vi "FuncVI-QueuePut.vi"(5 "InstanceRef":T2, 9 "arg list":T1[](array[typedef]) {"num" format="%.2f"}) -> (0 "error out":bool, 3 "result":T1 {"num" format="%.2f"})   [LabVIEW 2021]
doc: "::: CalcExpress Toolkit :::\nCopyright (c) 2000-2026 Konstantin Shifershteyn. All rights reserved."
uses:
  cetypes.llb/CalcExpress Function Argument Info.ctl
  cetypes.llb/CalcExpress Instance RefNum.ctl
panel:
  in  "max arg num":i32=4
  in  "min arg num":i32=2
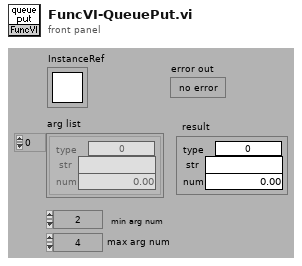
[diagram p1: front panel]
types:
  T1 = typedef "CalcExpress Function Argument Info.ctl" = cluster{"type":u32, "str":string, "num":dbl}
  T2 = typedef "CalcExpress Instance RefNum.ctl" = refnum<k1>
  T3 = cluster{"index":i32, "data type":enum32{"String", "DBL Number", "identifier", "1D Array of DBL", "2D Array of DBL", "CDB Number", "1D Array of CDB", "2D Array of CDB", "1D Array of String", "2D Array of String", "Unknown data type"}, "default num":dbl, "default str":string}[]
  T4 = enum32{"String", "DBL Number", "identifier", "1D Array of DBL", "2D Array of DBL", "CDB Number", "1D Array of CDB", "2D Array of CDB", "1D Array of String", "2D Array of String", "Unknown data type"}
  T5 = cluster{"data type":enum32{"String", "DBL Number", "identifier", "1D Array of DBL", "2D Array of DBL", "CDB Number", "1D Array of CDB", "2D Array of CDB", "1D Array of String", "2D Array of String", "Unknown data type"}, string, dbl}
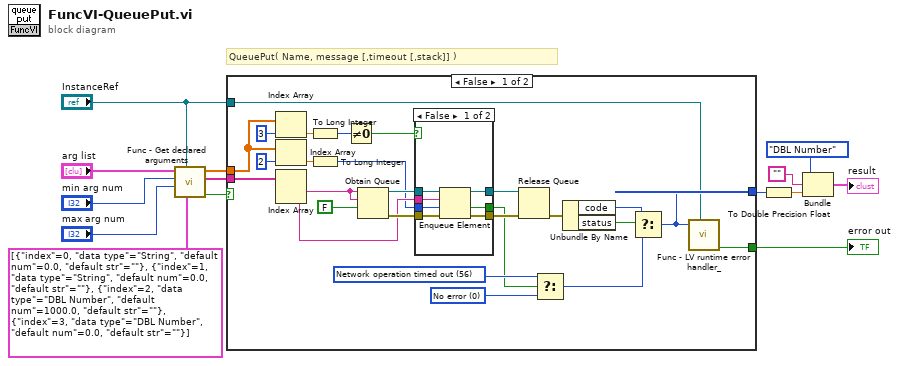
[diagram p0: block diagram]
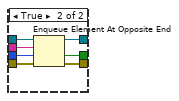
[diagram p2: hidden frame]
diagram:
  # "QueuePut( Name, message [,timeout [,stack]] )"
  n1 = call "Func - Get declared arguments.vi"("arg descriptors"=T3 [{"index"=0, "data type"=enum."String", "default num"=0.0, "default str"=""}, {"index"=1, "data type"=enum."String", "default num"=0.0, "default str"=""}, {"index"=2, "data type"=enum."DBL Number", "default num"=1000.0, "default str"=""}, {"index"=3, "data type"=enum."DBL Number", "default num"=0.0, "default str"=""}], "InstanceRef"="InstanceRef", "max arg num"="max arg num", "min arg num"="min arg num", "arg list"="arg list") -> ("error out"=w4:bool, "str list"=w13:string[], "num list"=w5:dbl[])  [unwired: 3 in, 1 out]
  n2 = case shown="False" w4 {
    selector: w4 -> [_ w55]
    tunnel: w13 -> [w40 _]
    tunnel: "InstanceRef" -> [w39 _]
    tunnel: [w27 _] -> w7
    tunnel: w5 -> [w36 _]
    tunnel: [w26 w55] -> w3
    frame False {
      w28 = 0 items=["No error", "Argument error", "Memory is full", "Out of zone", "End of file", "File already open", "Generic file I/O error", "File not found", "File permission error", "Disk is full", "Duplicate path", "Too many files open", "System feature not enabled", "Resource file not found", "Cannot add resource", "Resource not found", "Image not found", "Image memory error", "Pen does not exist", "Config type invalid", "Config token not found", "Config parse error", "Config memory error", "Bad external code format", "Bad external code offset", "External code not present", "Null window", "Destroy window error", "Null menu", "Print aborted", "Bad print record", "Print driver error", "Windows error during printing", "Memory error during printing", "Print dialog error", "Generic print error", "Invalid device refnum", "Device not found", "Device parameter error", "Device unit error", "Cannot open device", "Device call aborted", "Generic error", "Cancelled by user", "Object ID too low", "Object ID too high", "Object not in heap", "Unknown heap", "Unknown object (invalid DefProc)", "Unknown object (DefProc not in table)", "Message out of range", "Invalid (null) method", "Unknown message", "Manager call not supported", "Bad address", "Network operation in progress", "Network operation timed out", "Connection is busy", "Network attribute not supported", "Network error", "Address in use", "System out of memory", "Connection aborted", "Connection refused", "Not connected", "Already connected", "Connection closed", "Initialization error (interapplication manager)", "Bad occurrence", "Wait on unbound occurrence handler", "Occurrence queue overflow", "Datalog type conflict", "Unused", "Unrecognized type (interapplication manager)", "Memory corrupt", "Failed to make temporary DLL", "Old CIN version", "Drag socket not found", "Failed to load drop-object", "Failed to register OLE object", "Failed to release OLE object", "Format specifier type mismatch", "Unknown format specifier", "Too few format specifiers", "Too many format specifiers", "Scan failed", "Newer CIN version", "OLE Convert", "Runtime menu error", "Password tampered", "Unknown error code"]
      w31 = 56 items=["No error", "Argument error", "Memory is full", "Out of zone", "End of file", "File already open", "Generic file I/O error", "File not found", "File permission error", "Disk is full", "Duplicate path", "Too many files open", "System feature not enabled", "Resource file not found", "Cannot add resource", "Resource not found", "Image not found", "Image memory error", "Pen does not exist", "Config type invalid", "Config token not found", "Config parse error", "Config memory error", "Bad external code format", "Bad external code offset", "External code not present", "Null window", "Destroy window error", "Null menu", "Print aborted", "Bad print record", "Print driver error", "Windows error during printing", "Memory error during printing", "Print dialog error", "Generic print error", "Invalid device refnum", "Device not found", "Device parameter error", "Device unit error", "Cannot open device", "Device call aborted", "Generic error", "Cancelled by user", "Object ID too low", "Object ID too high", "Object not in heap", "Unknown heap", "Unknown object (invalid DefProc)", "Unknown object (DefProc not in table)", "Message out of range", "Invalid (null) method", "Unknown message", "Manager call not supported", "Bad address", "Network operation in progress", "Network operation timed out", "Connection is busy", "Network attribute not supported", "Network error", "Address in use", "System out of memory", "Connection aborted", "Connection refused", "Not connected", "Already connected", "Connection closed", "Initialization error (interapplication manager)", "Bad occurrence", "Wait on unbound occurrence handler", "Occurrence queue overflow", "Datalog type conflict", "Unused", "Unrecognized type (interapplication manager)", "Memory corrupt", "Failed to make temporary DLL", "Old CIN version", "Drag socket not found", "Failed to load drop-object", "Failed to register OLE object", "Failed to release OLE object", "Format specifier type mismatch", "Unknown format specifier", "Too few format specifiers", "Too many format specifiers", "Scan failed", "Newer CIN version", "OLE Convert", "Runtime menu error", "Password tampered", "Unknown error code"]
      n3 = Index Array(array=w36, index=3) -> (element=w35:dbl)
      n4 = Index Array(array=w36, index=2) -> (element=w34:dbl)
      n5 = Index Array(array=w40) -> (element #1=w18:string, element #2=w17:string)  [unwired: 2 in]
      n6 = To Long Integer(number=w35) -> (32bit integer=w33:i32)
      n7 = To Long Integer(number=w34) -> (32bit integer=w16:i32)
      n8 = Not Equal To 0?(x=w33) -> (x != 0?=w20:bool)
      n9 = Obtain Queue(name (unnamed)=w18, element data type=w18, create if not found? (T)=FALSE) -> (queue out=w25:refnum<queue>, error out=w23:errorcluster)  [unwired: 2 in, 1 out]
      n10 = case shown="False" w20 {
        tunnel: w25 -> [w47 w54]
        tunnel: [w46 w51] -> w24
        tunnel: w23 -> [w45 w53]
        tunnel: [w44 w52] -> w22
        tunnel: [w43 w50] -> w19
        tunnel: w17 -> [w42 w49]
        tunnel: w16 -> [w41 w48]
        frame False {
          n11 = Enqueue Element(queue=w47, element=w42, timeout in ms (-1)=w41, error in (no error)=w45) -> (queue out=w46:refnum<queue>, timed out?=w43:bool, error out=w44:errorcluster)
        }
        frame True {
          n12 = Enqueue Element At Opposite End(queue=w54, element=w49, timeout in ms (-1)=w48, error in (no error)=w53) -> (queue out=w51:refnum<queue>, timed out?=w50:bool, error out=w52:errorcluster)
        }
      }
      n13 = Release Queue(queue=w24, error in (no error)=w22) -> (error out=w15:errorcluster)  [unwired: 1 in, 2 out]
      n14 = Select(t=w31, s=w19, f=w28) -> (s? t:f=w32:i32)
      n15 = Unbundle By Name(w15) -> ("code"=w30:i32, "status"=w29:bool)
      n16 = Select(t=w30, s=w29, f=w32) -> (s? t:f=w27:i32)
      n17 = call "Func - LV runtime error handler_.vi"("InstanceRef"=w39, "LabVIEW error code"=w27) -> ("error out"=w26:bool)  [unwired: 9 in]
    }
    frame True {
    }
  }
  "error out" <- w3
  n18 = To Double Precision Float(number=w7) -> (double precision float=w12:dbl)
  n19 = Bundle("data type"=T4."DBL Number", "", w12) -> (→"result":T5)  [unwired: 1 in]
